vi "Destroy.vi"(8 "error in (no error)":errorcluster, 11 "handler in":refnum<class "String Handler.lvclass">) -> (0 "error out":errorcluster)   [LabVIEW 2018, in "GLog.lvlib" / "String Handler.lvclass"]
uses:
  String Handler.lvclass
  C:/Users/Colin/Documents/software_projects/labview/glog/src/api/extension/formatting_handler_interface/Formatting Handler.lvclass
  extension/formatting_handler_interface/Formatting Handler.lvclass/Formatting Handler.ctl
  UI Updater/UI Updater.lvlib
  extension/formatting_handler_interface/Formatting Handler.lvclass
panel:
  # "Connector Pane"
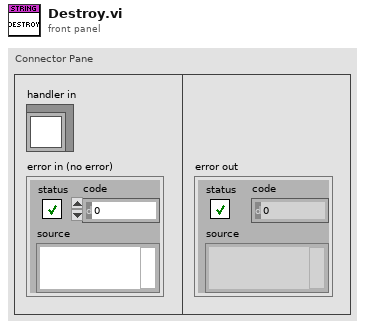
[diagram p1: front panel]
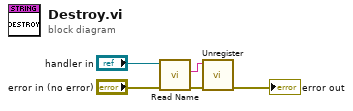
[diagram p0: block diagram]
diagram:
  n1 = call "Read Name.vi"("error in (no error)"="error in (no error)", "Formatting Handler in"="handler in") -> ("error out"=w1:errorcluster, "Name"=w2:string)  [unwired: 7 in, 1 out]
  n2 = call "Unregister.vi"("error in (no error)"=w1, "handler name"=w2) -> ("error out"=→"error out":errorcluster)  [unwired: 9 in]
